vi "Write FXP.vi"(6 "RegisterOffset":u32, 7 "FXP Configuration":T1, 8 "error in":errorcluster, 9 "DBL Value":dbl, 10 "register name":string, 11 "session in":u32) -> (0 "error out":errorcluster, 3 "session out":u32)   [LabVIEW 2020, in "FPGA Register IO.lvlib"]
uses:
  FPGA Register IO.lvlib
  TypeDefs/FXP Configuration.ctl
  <vilib>/fxp/LVFixedPointRepBitsTypeDef.ctl
  <vilib>/fxp/LVFixedPointRepRangeTypeDef.ctl
  Error Handling/Error 6006.vi
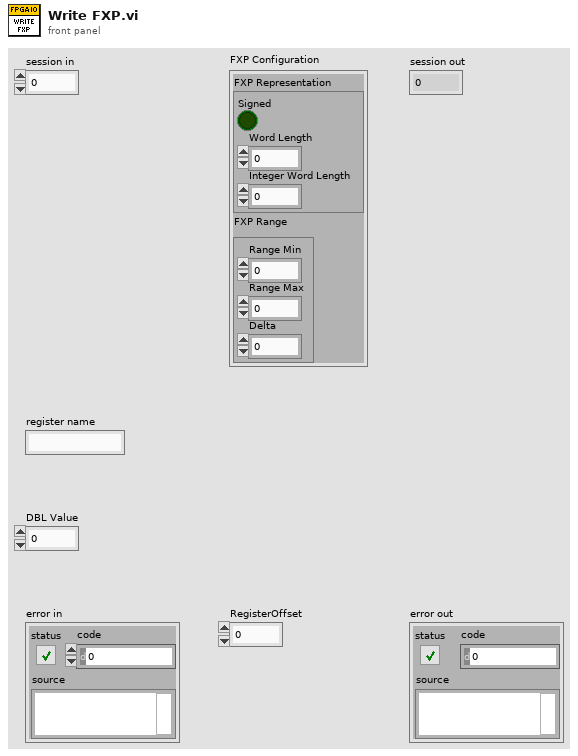
[diagram p1: front panel]
types:
  T1 = typedef "FPGA Register IO.lvlib/FXP Configuration.ctl" = cluster{"FXP Representation":T2, "FXP Range":T3}
  T2 = typedef "LVFixedPointRepBitsTypeDef.ctl" = cluster{"Signed":bool, "Word Length":u32, "Integer Word Length":i32}
  T3 = typedef "LVFixedPointRepRangeTypeDef.ctl" = cluster{"Range Min":dbl, "Range Max":dbl, "Delta":dbl}
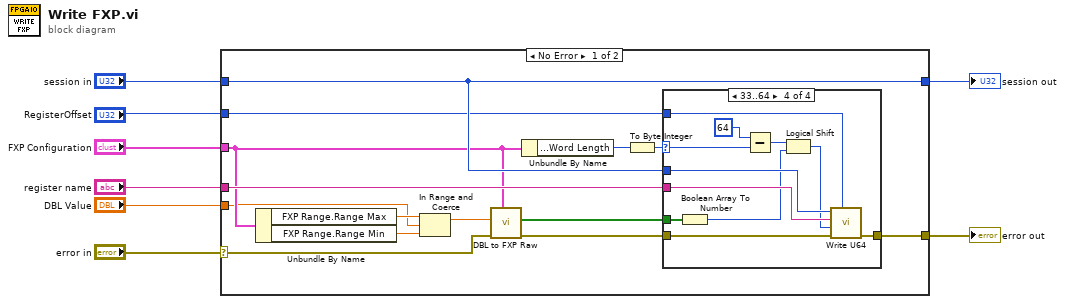
[diagram p0: block diagram]
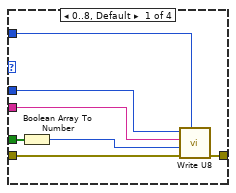
[diagram p2: hidden frame]
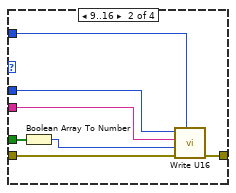
[diagram p3: hidden frame]
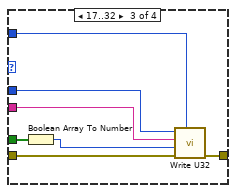
[diagram p4: hidden frame]
diagram:
  n1 = case shown="No Error" "error in" {
    selector: "error in" -> [w11 w56]
    tunnel: "session in" -> [w22 w55]
    tunnel: [w21 w56] -> w7
    tunnel: [w22 w55] -> w5
    tunnel: "FXP Configuration" -> [w16 _]
    tunnel: "DBL Value" -> [w13 _]
    tunnel: "register name" -> [w17 _]
    tunnel: "RegisterOffset" -> [w9 _]
    frame No Error {
      n2 = Unbundle By Name(w16) -> ("FXP Range.Range Max"=w15:dbl, "FXP Range.Range Min"=w14:dbl)
      n3 = In Range and Coerce(upper limit=w15, x=w13, lower limit=w14) -> (coerced(x)=w12:dbl)  [unwired: 1 out]
      n4 = call "DBL to FXP Raw.vi"("FXP Configuration"=w16, "error in (no error)"=w11, "DBL Value"=w12) -> ("error out"=w20:errorcluster, "Bool Data"=w19:bool[])  [unwired: 7 in]
      n5 = Unbundle By Name(w16) -> ("FXP Representation.Word Length"=w18:u32)
      n6 = To Byte Integer(number=w18) -> (8bit integer=w10:i8)
      n7 = case shown="33..64" w10 {
        selector: w10 -> [_ _ _ w47]
        tunnel: w22 -> [w28 w34 w41 w51]
        tunnel: w20 -> [w29 w36 w43 w54]
        tunnel: [w27 w35 w42 w53] -> w21
        tunnel: w19 -> [w26 w33 w40 w52]
        tunnel: w17 -> [w25 w32 w39 w50]
        tunnel: w9 -> [w24 w31 w38 w44]
        frame 0..8, Default {
          n8 = Boolean Array To Number(Boolean array=w26) -> (number=w23:u8)
          n9 = call "Write U8.vi"("RegisterOffset"=w24, "error in"=w29, "value in"=w23, "register name"=w25, "session in"=w28) -> ("error out"=w27:errorcluster)  [unwired: 5 in, 1 out]
        }
        frame 9..16 {
          n10 = Boolean Array To Number(Boolean array=w33) -> (number=w30:u16)
          n11 = call "Write U16.vi"("RegisterOffset"=w31, "error in"=w36, "value in"=w30, "register name"=w32, "session in"=w34) -> ("error out"=w35:errorcluster)  [unwired: 5 in, 1 out]
        }
        frame 17..32 {
          n12 = Boolean Array To Number(Boolean array=w40) -> (number=w37:u32)
          n13 = call "Write U32.vi"("RegisterOffset"=w38, "error in"=w43, "value in"=w37, "register name"=w39, "session in"=w41) -> ("error out"=w42:errorcluster)  [unwired: 5 in, 1 out]
        }
        frame 33..64 {
          n14 = Boolean Array To Number(Boolean array=w52) -> (number=w46:u64)
          n15 = Subtract(x=i8 64 ("y"), y=w47) -> (x-y=w48:i8)
          n16 = Logical Shift(y=w48, x=w46) -> (x << y=w45:u64)
          n17 = call "Write U64.vi"("RegisterOffset"=w44, "error in"=w54, "value in"=w45, "register name"=w50, "session in"=w51) -> ("error out"=w53:errorcluster)  [unwired: 5 in, 1 out]
        }
      }
    }
    frame Error {
    }
  }
  "error out" <- w7
  "session out" <- w5
